vi "Read FCC Part15c Default SA Setting.vi"(8 "error in (no error)":errorcluster, 11 "Band Edge in":refnum<class "Band Edge.lvclass">) -> (0 "error out":errorcluster, 2 "Cluster":T1 {"Frequency Line (Hz)"."Line 2" format="%#_6p"; "Frequency Line (Hz)"."Line 1" format="%#_6p"; "Marker Search Freq (Hz)"."Right Limit" format="%#_6p"; "Marker Search Freq (Hz)"."Left Limit" format="%#_6p"; "Sweep Time(sec)" format="%#_6p"; "VBW(Hz)" format="%#_6p"; "RBW(Hz)" format="%#_6p"; "Start/Stop Frequency(Hz)"."Stop" format="%#_6p"; "Start/Stop Frequency(Hz)"."Start" format="%#_6p"}, 3 "Band Edge out":refnum<class "Band Edge.lvclass">)   [LabVIEW 2023, in "Spectrum Analyzer.lvlib" / "Band Edge.lvclass"]
uses:
  Band Edge.lvclass
  Band Edge.lvclass/Band Edge.ctl
  TYPE DEFINITION/TYPE Start and Stop Frequency.ctl
  Spectrum Analyzer.lvlib
  TYPE DEFINITION/TYPE Display Trace Mode Select.ctl
  TYPE DEFINITION/TYPE Detect Mode Select.ctl
  TYPE DEFINITION/TYPE FCC Part15c Standard BandEdge Setting Cluster.ctl
  TYPE DEFINITION/TYPE Spectrum Window Select.ctl
  TYPE DEFINITION/TYPE Marker Search Limit Set.ctl
  TYPE DEFINITION/TYPE Frequency Line Param.ctl
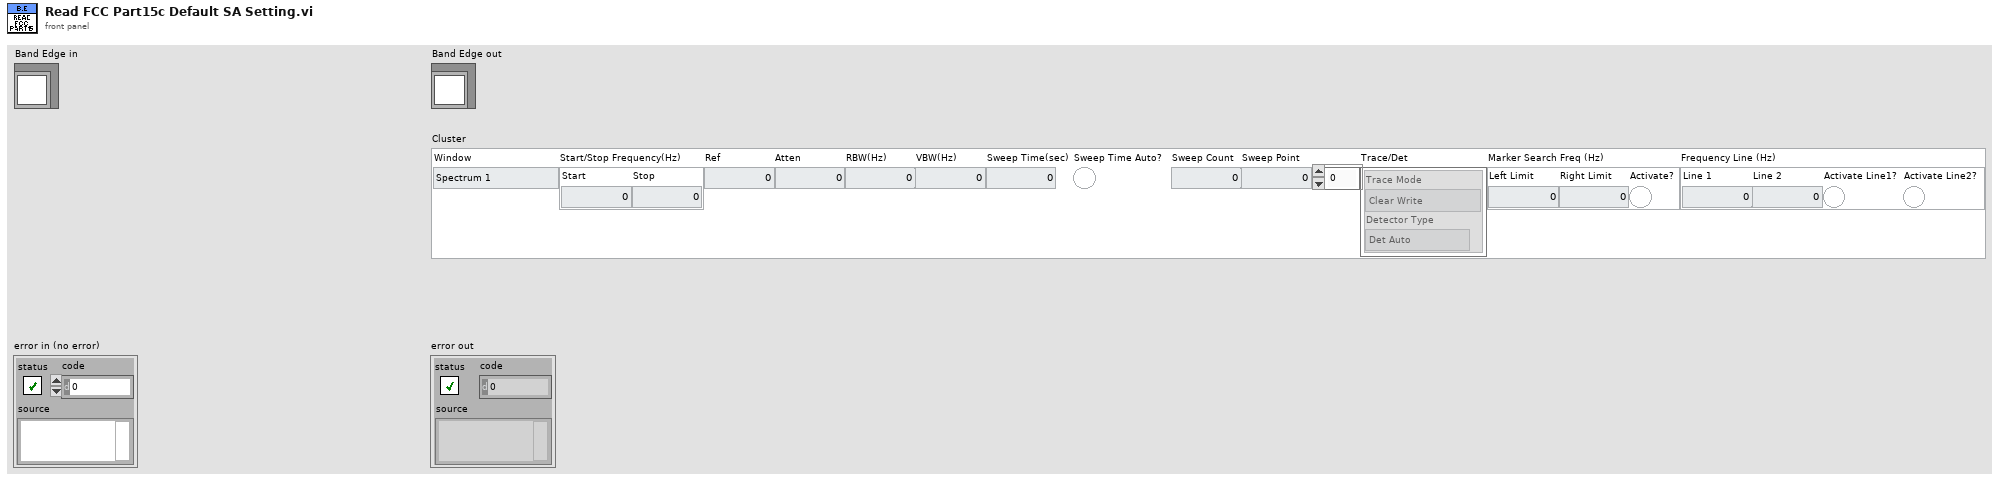
[diagram p1: front panel]
types:
  T1 = typedef "Spectrum Analyzer.lvlib/TYPE FCC Part15c Standard BandEdge Setting Cluster.ctl" = cluster{"Window":T2, "Start/Stop Frequency(Hz)":T3, "Ref":dbl, "Atten":i32, "RBW(Hz)":dbl, "VBW(Hz)":dbl, "Sweep Time(sec)":dbl, "Sweep Time Auto?":bool, "Sweep Count":u32, "Sweep Point":u32, "Trace/Det":cluster{"Trace Mode":T4, "Detector Type":T5}[], "Marker Search Freq (Hz)":T6, "Frequency Line (Hz)":T7}
  T2 = typedef "Spectrum Analyzer.lvlib/TYPE Spectrum Window Select.ctl" = enum16{"Spectrum 1", "Spectrum 2", "Spectrum 3", "Spectrum 4"}
  T3 = typedef "Spectrum Analyzer.lvlib/TYPE Start and Stop Frequency.ctl" = cluster{"Start":dbl, "Stop":dbl}
  T4 = typedef "Spectrum Analyzer.lvlib/TYPE Display Trace Mode Select.ctl" = enum16{"Clear Write", "Max Hold", "Min Hold", "Average", "View"}
  T5 = typedef "Spectrum Analyzer.lvlib/TYPE Detect Mode Select.ctl" = enum16{"Det Auto", "Auto Peak", "Positive Peak", "Negative Peak", "Sample", "RMS", "Average", "Quasipeak", "CISPR Average", "RMS Average"}
  T6 = typedef "Spectrum Analyzer.lvlib/TYPE Marker Search Limit Set.ctl" = cluster{"Left Limit":dbl, "Right Limit":dbl, "Activate?":bool}
  T7 = typedef "Spectrum Analyzer.lvlib/TYPE Frequency Line Param.ctl" = cluster{"Line 1":dbl, "Line 2":dbl, "Activate Line1?":bool, "Activate Line2?":bool}
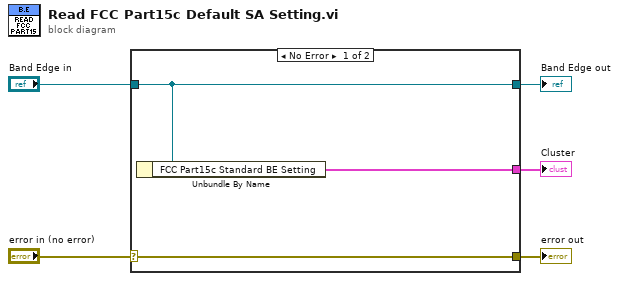
[diagram p0: block diagram]
diagram:
  n1 = case shown="No Error" "error in (no error)" {
    selector: "error in (no error)" -> [w8 w9]
    tunnel: [w8 w9] -> w4
    tunnel: [w7 w10] -> w2
    tunnel: "Band Edge in" -> [w7 w10]
    tunnel: [w6 _] -> w1
    frame No Error {
      n2 = Unbundle By Name(w7) -> ("FCC Part15c Standard BE Setting"=w6:T1)
    }
    frame Error {
    }
  }
  "error out" <- w4
  "Band Edge out" <- w2
  "Cluster" <- w1
